vi "Set_Output.vi"(8 "error in (no error)":errorcluster, 10 "Output":dbl, 11 "object in":refnum<class "AIO_Channel.lvclass">) -> (0 "error out":errorcluster, 3 "object out":refnum<class "AIO_Channel.lvclass">)   [LabVIEW 2021, in "Simulator-Channel.lvlib" / "AIO_Channel.lvclass"]
doc: "Sets the Digital Output"
uses:
  AIO_Channel.lvclass
  C:/Users/averna/Documents/LV Gym DEMO/Factory Pattern/Device Channels/Dependencies/AIO-Channel.lvlibp/Channels/AIO-Channel/AIO_Channel_class/AIO_Channel.lvclass
  AIO_Channel.lvclass/AIO_Channel.ctl
  AIO_Panel/DIO_Panel Messages/Set Output Msg/Set Output Msg.lvclass/Set Output Msg.ctl
  <vilib>/ActorFramework/Message Enqueuer/Message Enqueuer.lvclass/Message Enqueuer.ctl
  <vilib>/ActorFramework/Message Enqueuer/Enqueue.vi
  AIO_Panel/DIO_Panel Messages/Set Output Msg/Set Output Msg.lvclass
  C:/Program Files/National Instruments/LabVIEW 2021/vi.lib/ActorFramework/Message/Message.lvclass
  Dependencies/AIO-Channel.lvlibp/Channels/AIO-Channel/AIO_Channel_class/Properties/GetAIOConfiguration.vi
  <vilib>/ActorFramework/Message Priority Queue/Priority Enqueue.vi
  Dependencies/AIO-Channel.lvlibp/Channels/AIO-Channel/AIO-Configuration_class/AIO-Configuration.lvclass
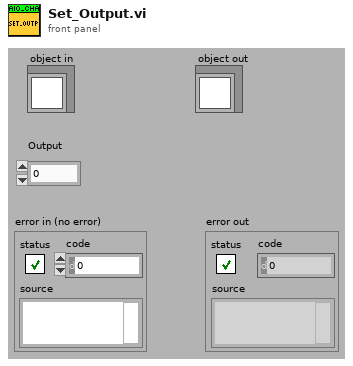
[diagram p1: front panel]
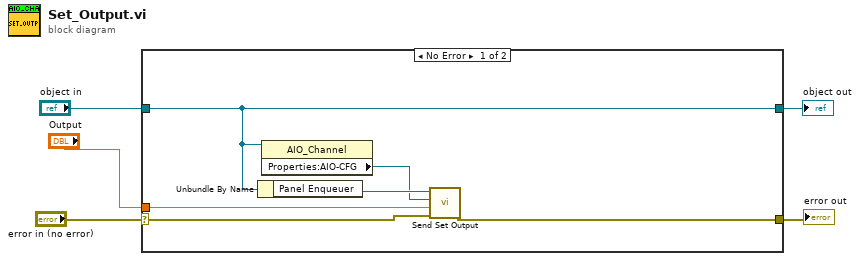
[diagram p0: block diagram]
diagram:
  n1 = case shown="No Error" "error in (no error)" {
    selector: "error in (no error)" -> [w8 w13]
    tunnel: [w7 w13] -> w4
    tunnel: [w9 w12] -> w2
    tunnel: "object in" -> [w9 w12]
    tunnel: "Output" -> [w6 _]
    frame No Error {
      n2 = Unbundle By Name(w9) -> ("Panel Enqueuer"=w11:refnum<class "Message Enqueuer.lvclass">)
      n3 = property class="AIO_Channel"(reference=w9) -> ("Properties:AIO-CFG"=w10:refnum<class "AIO-Configuration.lvclass">)  [unwired: 1 in, 2 out]
      n4 = call "Send Set Output.vi"("error in (no error)"=w8, "Set Output"=w6, "DIO_CFG"=w10, "Message Enqueuer"=w11) -> ("error out"=w7:errorcluster)  [unwired: 6 in, 1 out]
    }
    frame Error {
    }
  }
  "error out" <- w4
  "object out" <- w2
